vi "Share in Browser.vi"   [LabVIEW 2020]
doc: "Menu entry Tools > RemoteVI > Share in Browser. Opens RemoteVI Server and closes its own window."
uses:
  RemoteVI.lvlib
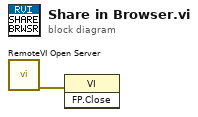
[diagram p0: block diagram]
diagram:
  n1 = call "RemoteVI Open Server.vi"() -> ("error out"=w1:errorcluster)  [unwired: 15 in]
  n2 = invoke class="VI" method="FP.Close"(error in=w1) -> ()  [unwired: 2 in, 3 out]
